vi "Measure.vi"(8 "error in (no error)":errorcluster, 9 "measurement configuration":variant, 10 "measure call context in":refnum<class "Measure Call Context.lvclass">, 11 "measurement plugin in":refnum<class "CAN-LIN Raw Bus Capture.lvclass">) -> (0 "error out":errorcluster, 1 "measurement results":variant, 2 "measure call context out":refnum<class "Measure Call Context.lvclass">, 3 "measurement plugin out":refnum<class "CAN-LIN Raw Bus Capture.lvclass">)   [LabVIEW 2025, in "CAN-LIN Raw Bus Capture.lvclass"]
uses:
  CAN-LIN Raw Bus Capture.lvclass
  <vilib>/Plug-In SDKs/Measurements/Measure Call Context/Measure Call Context.lvclass
  Measurement Configuration.ctl
  CAN-LIN Raw Bus Capture.lvclass/CAN-LIN Raw Bus Capture.ctl
  CAN-LIN Raw Bus Capture UI/Toggle.ctl
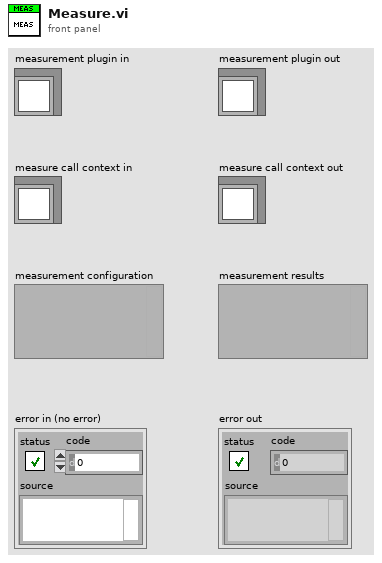
[diagram p1: front panel]
types:
  T1 = typedef "CAN-LIN Raw Bus Capture.lvclass/Measurement Configuration.ctl" = cluster{"INTERFACE NAME CAN":refnum<k21>, "Termination CAN":T2, "FD Baudrate":u32, "Baudrate":u32, "FD ISO Mode":enum16{"ISO", "Legacy ISO", "Non-ISO"}, "IO Mode":enum16{"CAN", "CAN FD", "CAN FD + BRS"}, "SortByID":bool, "Filter":string, "INTERFACE NAME LIN":refnum<k21>, "Termination LIN":T2}
  T2 = typedef "Toggle.ctl" = bool
  T3 = typedef "CAN-LIN Raw Bus Capture.lvclass/Measurement Results.ctl" = cluster{"CAN Bus Info":string, "Display":string[][]}
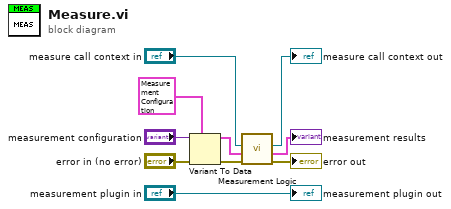
[diagram p0: block diagram]
diagram:
  n1 = Variant To Data(error in="error in (no error)", type=T1 {"INTERFACE NAME CAN"="", "Termination CAN"=FALSE, "FD Baudrate"=1, "Baudrate"=32, "FD ISO Mode"=enum."Non-ISO", "IO Mode"=enum."CAN FD + BRS", "SortByID"=FALSE, "Filter"="", "INTERFACE NAME LIN"="", "Termination LIN"=FALSE} ("measurement configuration"), Variant="measurement configuration") -> (data=w1:T1, error out=w7:errorcluster)
  n2 = call "Measurement Logic.vi"("error in"=w7, "measurement configuration"=w1, "measure call context in"="measure call context in") -> ("error out"=→"error out":errorcluster, "measurement results"=→"measurement results":T3, "measure call context out"=→"measure call context out":refnum<class "Measure Call Context.lvclass">)  [unwired: 6 in]
  "measurement plugin out" <- "measurement plugin in"
